vi "FRC Copy Project.vi"(0 "source project folder":path, 5 "target path":path, 7 "original project name":string, 9 "new project name":string, 11 "error in":errorcluster) -> (4 "new project path":path, 15 "error out":errorcluster)   [LabVIEW 2025]
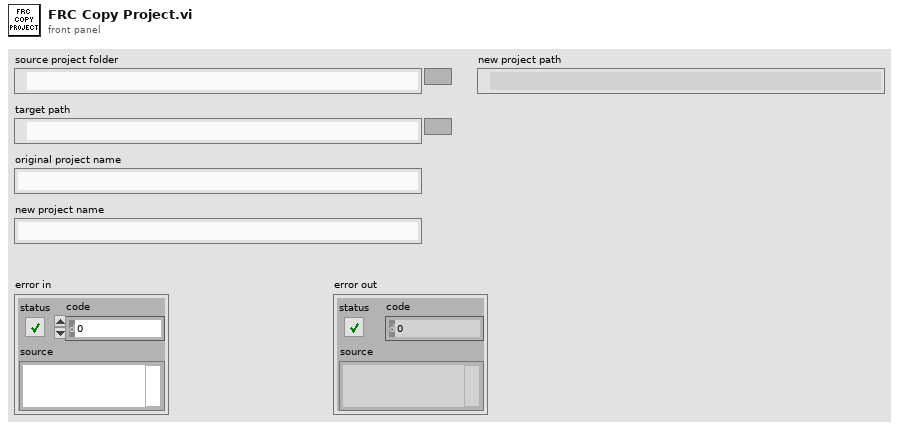
[diagram p1: front panel]
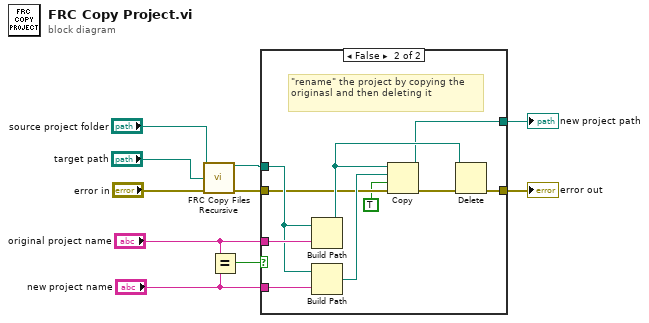
[diagram p0: block diagram]
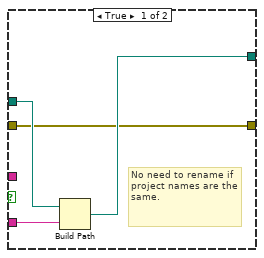
[diagram p2: hidden frame]
diagram:
  n1 = call "FRC Copy Files Recursive.vi"("source project folder"="source project folder", "target project folder"="target path", "error in"="error in") -> ("target path out"=w1:path)  [unwired: 11 in, 1 out]
  n2 = Equal?(x="original project name", y="new project name") -> (x = y?=w5:bool)
  n3 = case shown="False" w5 {
    tunnel: "original project name" -> [_ w23]
    tunnel: "new project name" -> [w13 w22]
    tunnel: [w10 w18] -> w9
    tunnel: [w11 w17] -> w8
    tunnel: w1 -> [w12 w16]
    tunnel: "error in" -> [w10 w15]
    frame True {
      # "No need to rename if project names are the same."
      n4 = Build Path(base path=w12, name or relative path=w13) -> (appended path=w11:path)
    }
    frame False {
      # "\"rename\" the project by copying the originasl and then deleting it"
      n5 = Build Path(base path=w16, name or relative path=w23) -> (appended path=w19:path)
      n6 = Build Path(base path=w16, name or relative path=w22) -> (appended path=w21:path)
      n7 = Copy(8:w15, 9:TRUE ("overwrite (F)"), 10:w21, 11:w19) -> (0:w20:errorcluster, 3:w17:path)  [unwired: 1 in, 1 out]
      n8 = Delete(path (use dialog)=w19, error in=w20) -> (error out=w18:errorcluster)  [unwired: 3 in, 2 out]
    }
  }
  "error out" <- w9
  "new project path" <- w8
